vi "Calculate angle.vi"(10 "XY Coordinates":i32[](array[numeric])) -> (1 "Angle (deg)":dbl)   [LabVIEW 2020]
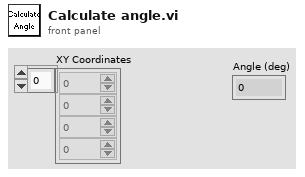
[diagram p1: front panel]
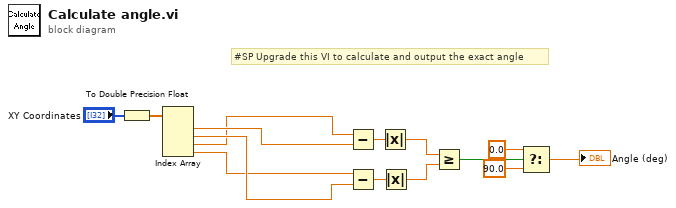
[diagram p0: block diagram]
diagram:
  # "#SP Upgrade this VI to calculate and output the exact angle"
  n1 = To Double Precision Float(number="XY Coordinates") -> (double precision float=w4:dbl[])
  n2 = Index Array(array=w4) -> (element #1=w9:dbl, element #2=w8:dbl, element #3=w7:dbl, element #4=w6:dbl)  [unwired: 4 in]
  n3 = Subtract(x=w7, y=w9) -> (x-y=w12:dbl)
  n4 = Subtract(x=w6, y=w8) -> (x-y=w13:dbl)
  n5 = Absolute Value(x=w12) -> (abs(x)=w11:dbl)
  n6 = Absolute Value(x=w13) -> (abs(x)=w10:dbl)
  n7 = Greater Or Equal?(x=w11, y=w10) -> (x >= y?=w3:bool)
  n8 = Select(t=0.0, s=w3, f=90.0) -> (s? t:f=→"Angle (deg)":dbl)
